vi "Heater Control.vi"(8 "error in":errorcluster, 11 "LNG Boiling Results in":refnum<class "LNG Boiling Results.lvclass">) -> (0 "error out":errorcluster, 2 "Htr MOS Ctrl":dbl, 3 "LNG Boiling Results out":refnum<class "LNG Boiling Results.lvclass">)   [LabVIEW 2019, in "Results.lvlib" / "LNG Boiling Results.lvclass"]
uses:
  LNG Boiling Results.lvclass
  LNG Boiling Results.lvclass/LNG Boiling Results.ctl
  <vilib>/gmath/NI_Gmath.lvlib
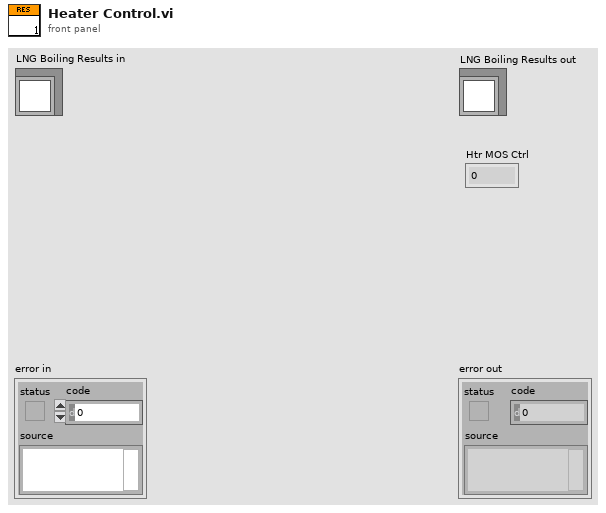
[diagram p1: front panel]
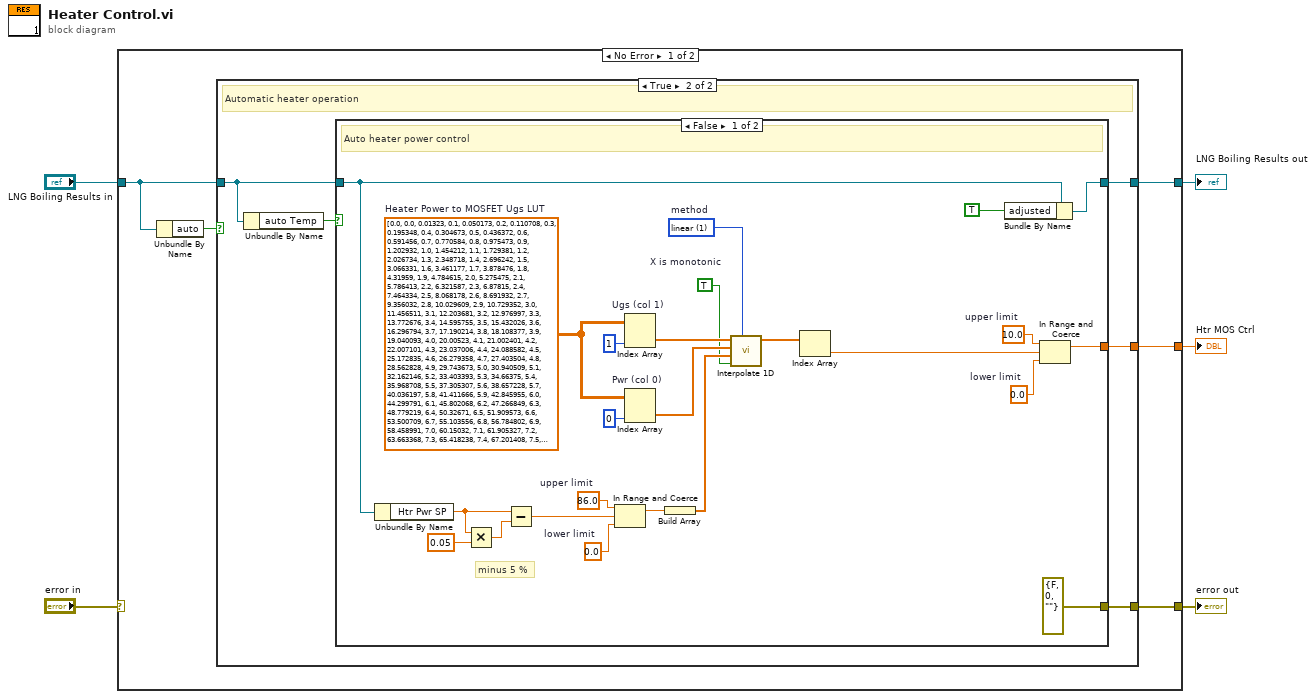
[diagram p0: block diagram]
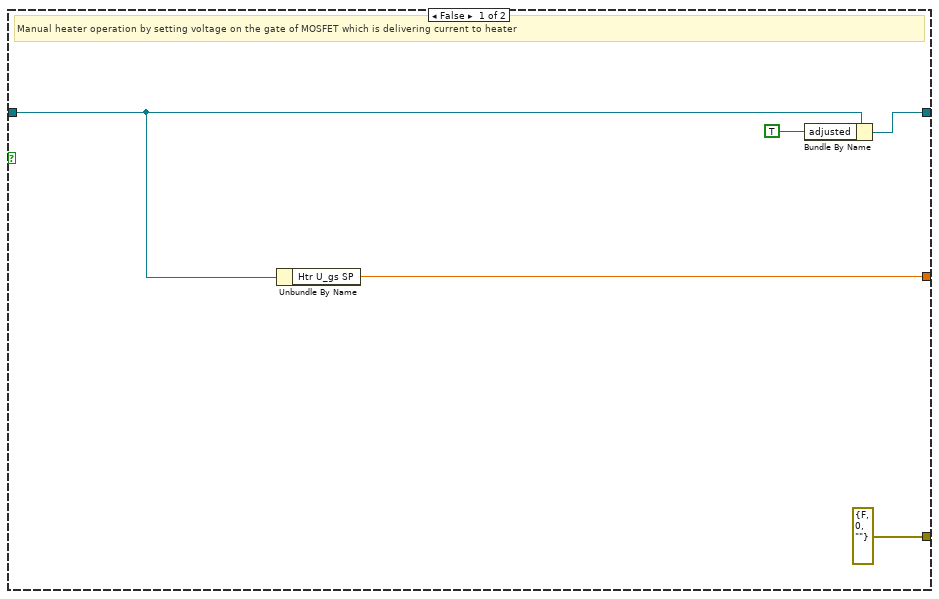
[diagram p2: hidden frame]
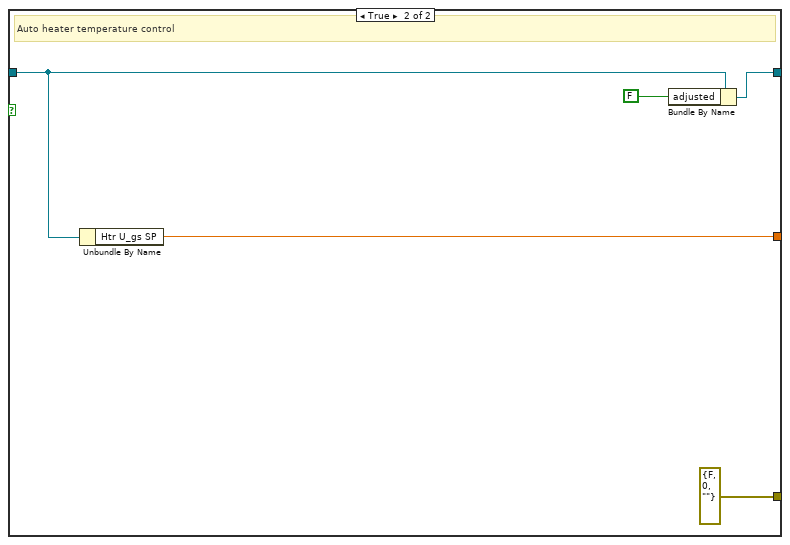
[diagram p3: hidden frame]
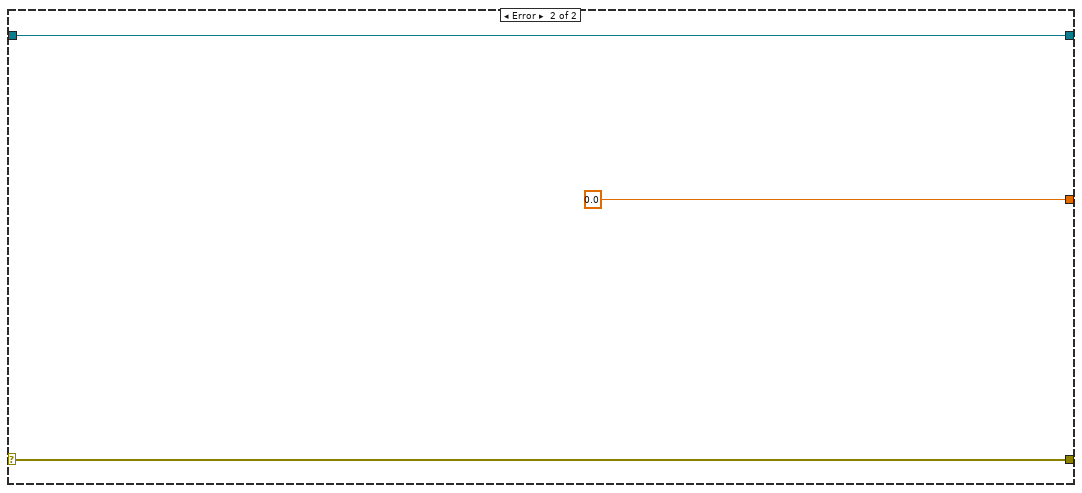
[diagram p4: hidden frame]
diagram:
  n1 = case shown="No Error" "error in" {
    selector: "error in" -> [_ w52]
    tunnel: [w7 w52] -> w4
    tunnel: "LNG Boiling Results in" -> [w9 w50]
    tunnel: [w10 0.0 ("Htr MOS Ctrl")] -> w2
    tunnel: [w6 w50] -> w1
    frame No Error {
      n2 = Unbundle By Name(w9) -> ("auto"=w8:bool)
      n3 = case shown="True" w8 {
        tunnel: [w11 w18] -> w10
        tunnel: w9 -> [w14 w20]
        tunnel: [errorcluster {"status"=FALSE, "code"=0, "source"=""} ("error IO") w17] -> w7
        tunnel: [w12 w16] -> w6
        frame False {
          # "Manual heater operation by setting voltage on the gate of MOSFET which is delivering current to heater"
          n4 = Unbundle By Name(w14) -> ("Htr U_gs SP"=w11:dbl)
          n5 = Bundle By Name(cluster=w14, "adjusted"=TRUE) -> (w12:refnum<class "LNG Boiling Results.lvclass">)
        }
        frame True {
          # "Automatic heater operation"
          n6 = Unbundle By Name(w20) -> ("auto Temp"=w19:bool)
          n7 = case shown="False" w19 {
            tunnel: w20 -> [w41 w48]
            tunnel: [w31 w45] -> w18
            tunnel: [errorcluster {"status"=FALSE, "code"=0, "source"=""} ("error IO") errorcluster {"status"=FALSE, "code"=0, "source"=""} ("error IO")] -> w17
            tunnel: [w43 w47] -> w16
            frame False {
              w24 = 86.0  # upper limit
              w23 = 0.0  # lower limit
              w29 = 10.0  # upper limit
              w30 = 0.0  # lower limit
              w32 = TRUE  # X is monotonic
              w37 = dbl[][] [[0.0, 0.0], [0.01323, 0.1], [0.050173, 0.2], [0.110708, 0.3], [0.195348, 0.4], [0.304673, 0.5], [0.436372, 0.6], [0.591456, 0.7], [0.770584, 0.8], [0.975473, 0.9], [1.202932, 1.0], [1.454212, 1.1], [1.729381, 1.2], [2.026734, 1.3], [2.348718, 1.4], [2.696242, 1.5], [3.066331, 1.6], [3.461177, 1.7], [3.878476, 1.8], [4.31959, 1.9], [4.784615, 2.0], [5.275475, 2.1], [5.786413, 2.2], [6.321587, 2.3], [6.87815, 2.4], [7.464334, 2.5], [8.068178, 2.6], [8.691932, 2.7], [9.356032, 2.8], [10.029609, 2.9], [10.729352, 3.0], [11.456511, 3.1], [12.203681, 3.2], [12.976997, 3.3], [13.772676, 3.4], [14.595755, 3.5], [15.432026, 3.6], [16.296794, 3.7], [17.190214, 3.8], [18.108377, 3.9], [19.040093, 4.0], [20.00523, 4.1], [21.002401, 4.2], [22.007101, 4.3], [23.037006, 4.4], [24.088582, 4.5], [25.172835, 4.6], [26.279358, 4.7], [27.403504, 4.8], [28.562828, 4.9], [29.743673, 5.0], [30.940509, 5.1], [32.162146, 5.2], [33.403393, 5.3], [34.66375, 5.4], [35.968708, 5.5], [37.305307, 5.6], [38.657228, 5.7], [40.036197, 5.8], [41.411666, 5.9], [42.845955, 6.0], [44.299791, 6.1], [45.802068, 6.2], [47.266849, 6.3], [48.779219, 6.4], [50.32671, 6.5], [51.909573, 6.6], [53.500709, 6.7], [55.103556, 6.8], [56.784802, 6.9], [58.458991, 7.0], [60.15032, 7.1], [61.905327, 7.2], [63.663368, 7.3], [65.418238, 7.4], [67.201408, 7.5], [69.047424, 7.6], [70.888713, 7.7], [72.769718, 7.8], [74.65409, 7.9], [76.609252, 8.0], [78.64176, 8.1], [80.730287, 8.2], [82.801904, 8.3], [84.94474, 8.4], [85.23019, 8.5]]  # Heater Power to MOSFET Ugs LUT
              w40 = 1 items=["nearest", "linear", "spline", "cubic Hermite", "Lagrange"]  # method
              # "minus 5 %"
              # "Auto heater power control"
              n8 = Unbundle By Name(w41) -> ("Htr Pwr SP"=w26:dbl)
              n9 = Multiply(x=w26, y=0.05) -> (x*y=w27:dbl)
              n10 = Subtract(x=w26, y=w27) -> (x-y=w22:dbl)
              n11 = In Range and Coerce(upper limit=w24, x=w22, lower limit=w23) -> (coerced(x)=w21:dbl)  [unwired: 1 out]
              n12 = Index Array "Ugs (col 1)"(array=w37, index (col)=1 ("disabled index (col)")) -> (element=w36:dbl[])  [unwired: 1 in]
              n13 = Index Array "Pwr (col 0)"(array=w37, index (col)=0 ("disabled index (col)")) -> (element=w35:dbl[])  [unwired: 1 in]
              n14 = Build Array(w21) -> (w34:dbl[])
              n15 = call <vilib>:"Interpolate 1D.vi"("method"=w40, "X is monotonic"=w32, "xi"=w34, "X"=w35, "Y"=w36) -> ("yi"=w33:dbl[])  [unwired: 4 in, 2 out]
              n16 = Index Array(array=w33) -> (element=w25:dbl)  [unwired: 1 in]
              n17 = Bundle By Name(cluster=w41, "adjusted"=TRUE) -> (w43:refnum<class "LNG Boiling Results.lvclass">)
              n18 = In Range and Coerce(upper limit=w29, x=w25, lower limit=w30) -> (coerced(x)=w31:dbl)  [unwired: 1 out]
            }
            frame True {
              # "Auto heater temperature control"
              n19 = Unbundle By Name(w48) -> ("Htr U_gs SP"=w45:dbl)
              n20 = Bundle By Name(cluster=w48, "adjusted"=FALSE) -> (w47:refnum<class "LNG Boiling Results.lvclass">)
            }
          }
        }
      }
    }
    frame Error {
    }
  }
  "error out" <- w4
  "Htr MOS Ctrl" <- w2
  "LNG Boiling Results out" <- w1
